vi "Update Command.vi"(6 "Time":dbl, 8 "error in (no error)":errorcluster, 11 "2WayValve in":refnum<class "2WayValveH.lvclass">) -> (0 "error out":errorcluster, 3 "2WayValve out":refnum<class "2WayValveH.lvclass">)   [LabVIEW 2020, in "VolatusGUIElements.lvlib" / "2WayValveH.lvclass"]
uses:
  2WayValveH.lvclass
  2WayValveH.lvclass/2WayValveH.ctl
  lv-vecto/Vecto/Channel DBL/Channel DBL.lvclass/Channel DBL.ctl
  lv-vecto/Vecto/Group DBL/Value by Index.vi
  lv-vecto/Vecto/Channel DBL/Channel DBL.lvclass
  lv-vecto/Vecto/Vecto.lvlib
  VolatusGUIElements.lvlib
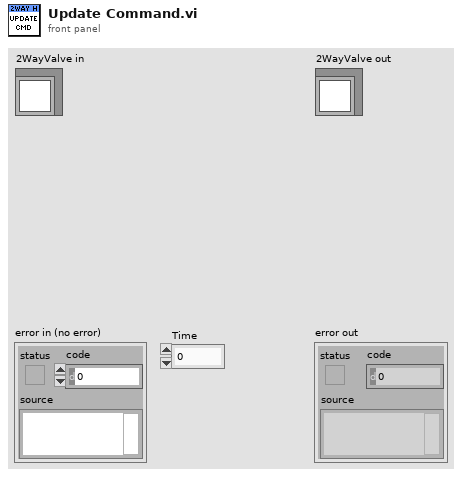
[diagram p1: front panel]
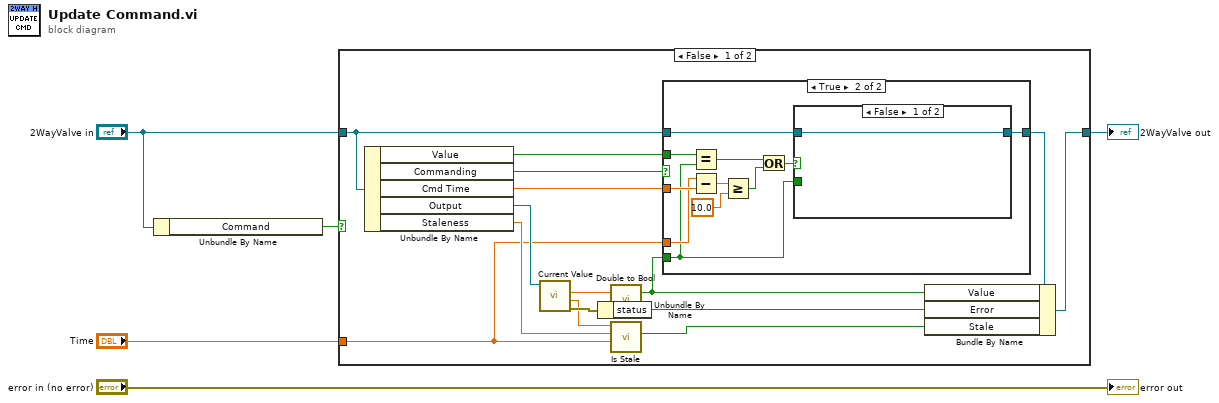
[diagram p0: block diagram]
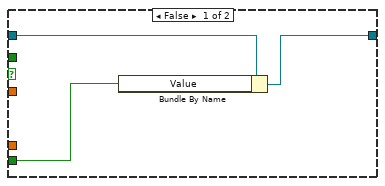
[diagram p2: hidden frame]
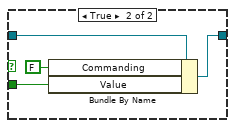
[diagram p3: hidden frame]
diagram:
  n1 = Unbundle By Name("2WayValve in") -> ("Command"=w4:bool)
  n2 = case shown="False" w4 {
    tunnel: [w6 w40] -> w3
    tunnel: "2WayValve in" -> [w7 w40]
    tunnel: "Time" -> [w9 _]
    frame False {
      n3 = Unbundle By Name(w7) -> ("Value"=w14:bool, "Commanding"=w16:bool, "Cmd Time"=w15:dbl, "Output"=w19:refnum<class "Channel DBL.lvclass">, "Staleness"=w10:dbl)
      n4 = call "Current Value.vi"("Channel in"=w19) -> ("error out"=w20:errorcluster, "Timestamp"=w11:dbl, "Scaled"=w18:dbl)  [unwired: 6 in, 2 out]
      n5 = Unbundle By Name(w20) -> ("status"=w17:bool)
      n6 = call "Double to Bool.vi"("Double"=w18) -> ("Bool"=w13:bool)  [unwired: 2 in]
      n7 = call "Is Stale.vi"("Time"=w9, "Staleness"=w10, "Timestamp"=w11) -> ("Stale"=w8:bool)  [unwired: 8 in]
      n8 = case shown="True" w16 {
        tunnel: w15 -> [_ w34]
        tunnel: w14 -> [_ w32]
        tunnel: w9 -> [_ w33]
        tunnel: w7 -> [w23 w27]
        tunnel: w13 -> [w21 w24]
        tunnel: [w22 w26] -> w12
        frame False {
          n9 = Bundle By Name(cluster=w23, "Value"=w21) -> (w22:refnum<class "2WayValveH.lvclass">)
        }
        frame True {
          n10 = Equal?(x=w32, y=w24) -> (x = y?=w31:bool)
          n11 = Subtract(x=w33, y=w34) -> (x-y=w30:dbl)
          n12 = Greater Or Equal?(x=w30, y=10.0) -> (x >= y?=w28:bool)
          n13 = Or(x=w31, y=w28) -> (x .or. y?=w25:bool)
          n14 = case shown="False" w25 {
            tunnel: w27 -> [w35 w39]
            tunnel: [w35 w38] -> w26
            tunnel: w24 -> [_ w36]
            frame False {
            }
            frame True {
              n15 = Bundle By Name(cluster=w39, "Commanding"=FALSE, "Value"=w36) -> (w38:refnum<class "2WayValveH.lvclass">)
            }
          }
        }
      }
      n16 = Bundle By Name(cluster=w12, "Value"=w13, "Error"=w17, "Stale"=w8) -> (w6:refnum<class "2WayValveH.lvclass">)
    }
    frame True {
      # "Command Unused"
    }
  }
  "2WayValve out" <- w3
  "error out" <- "error in (no error)"
